vi "subCheckPathAndName.vi"(4 "exclude instances?":bool, 6 "parent path":path, 10 "delimited name":string, 11 "path":path) -> (2 "path out":path, 3 "path to check?":bool)   [LabVIEW 2020, in "DependencyInspection.lvlib" / "CDependencyList.lvclass"]
uses:
  CDependencyList.lvclass
  CommonHelpers/CommonHelpers.lvlib
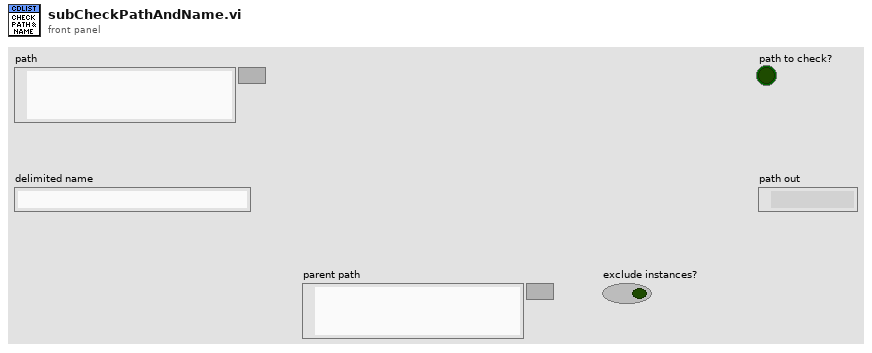
[diagram p1: front panel]
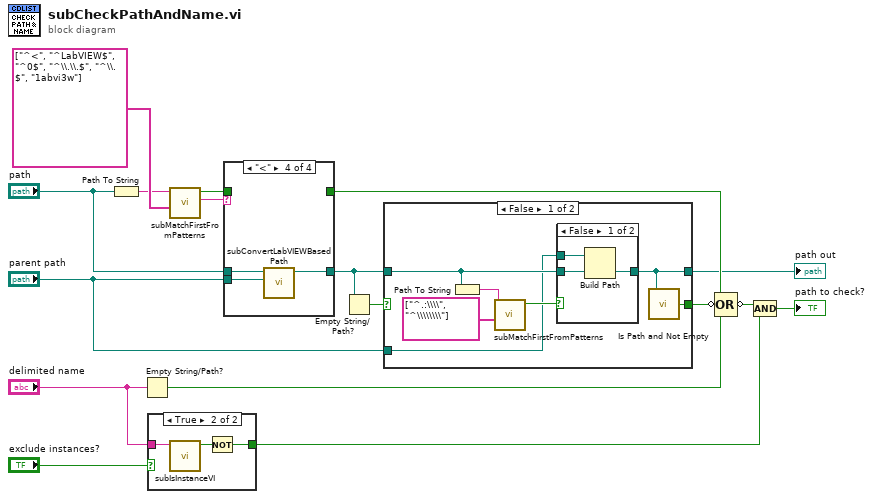
[diagram p0: block diagram]
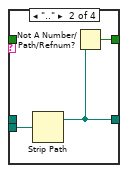
[diagram p5: hidden frame]
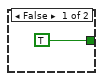
[diagram p7: hidden frame]
diagram:
  n1 = Path To String(path="path") -> (string=w8:string)
  n2 = Empty String/Path?(string/path="delimited name") -> (empty?=w17:bool)
  n3 = case shown="True" "exclude instances?" {
    tunnel: [TRUE w19] -> w16
    tunnel: "delimited name" -> [_ w20]
    frame False {
    }
    frame True {
      n4 = call "subIsInstanceVI.vi"("delimited name"=w20) -> ("found?"=w21:bool)  [unwired: 10 in]
      n5 = Not(x=w21) -> (.not. x?=w19:bool)
    }
  }
  n6 = call "subMatchFirstFromPatterns.vi"("patterns"=string[] ["^<", "^LabVIEW$", "^0$", "^\\.\\.$", "^\\.$", "1abvi3w"], "string in"=w8) -> ("matched string"=w11:string, "found?"=w9:bool)  [unwired: 7 in, 1 out]
  n7 = case shown="\"<\"" w11 {
    tunnel: [w23 w25 _ _] -> w10
    tunnel: w9 -> [w23 _ _ _]
    tunnel: "parent path" -> [_ w26 w27 w29]
    tunnel: "path" -> [w22 _ _ w30]
    tunnel: [w22 w24 w27 w28] -> w3
    frame Default {
    }
    frame ".." {
      n8 = Strip Path(path=w26) -> (stripped path=w24:path)  [unwired: 1 out]
      n9 = Not A Number/Path/Refnum?(number/path/refnum=w24) -> (NaN/Path/Refnum?=w25:bool)
    }
    frame "." {
    }
    frame "<" {
      n10 = call "subConvertLabVIEWBasedPath.vi"("Parent"=w29, "Path in"=w30) -> ("Path"=w28:path)  [unwired: 9 in]
    }
  }
  n11 = Empty String/Path?(string/path=w3) -> (empty?=w6:bool)
  n12 = case shown="False" w6 {
    selector: w6 -> [_ w43]
    tunnel: [w32 w43] -> w5
    tunnel: [w33 w42] -> w4
    tunnel: w3 -> [w34 w42]
    tunnel: "parent path" -> [w31 _]
    frame False {
      n13 = Path To String(path=w34) -> (string=w37:string)
      n14 = call "subMatchFirstFromPatterns.vi"("patterns"=string[] ["^.:\\\\", "^\\\\\\\\"], "string in"=w37) -> ("found?"=w35:bool)  [unwired: 7 in, 2 out]
      n15 = case shown="False" w35 {
        tunnel: w34 -> [w39 w41]
        tunnel: w31 -> [w40 _]
        tunnel: [w38 w41] -> w33
        frame False {
          n16 = Build Path(base path=w40, name or relative path=w39) -> (appended path=w38:path)
        }
        frame True {
        }
      }
      n17 = call <vilib>:"Is Path and Not Empty.vi"("path"=w33) -> ("Is Path and Not Empty?"=w32:bool)  [unwired: 4 in]
    }
    frame True {
    }
  }
  "path out" <- w4
  n18 = Compound Arithmetic op=OR(w10, invert w5, w17) -> (invert w1:bool)
  n19 = Compound Arithmetic op=AND(w1, w16) -> (→"path to check?":bool)
